vi "IO.vi"() -> ()   [LabVIEW 2024]
panel:
  in  "IO 16":bool
  in  "IO 15":bool
  in  "IO 14":bool
  in  "IO 13":bool
  in  "IO 12":bool
  in  "IO 11":bool
  in  "IO 10":bool
  in  "IO 9":bool
  in  "IO 8":bool
  in  "IO 7":bool
  in  "IO 6":bool
  in  "IO 5":bool
  in  "IO 4":bool
  in  "IO 3":bool
  in  "IO 2":bool
  in  "IO 1":bool
  out "IP":string="192.168.149.128"
  out "Port":dbl
  in  "Send":bool
  # "IO Light Control"
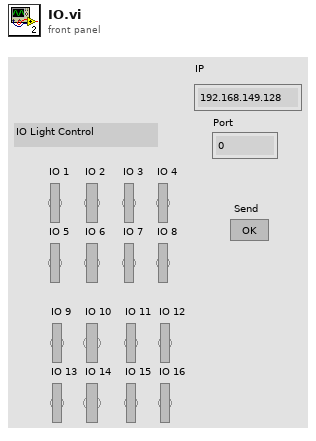
[diagram p1: front panel]
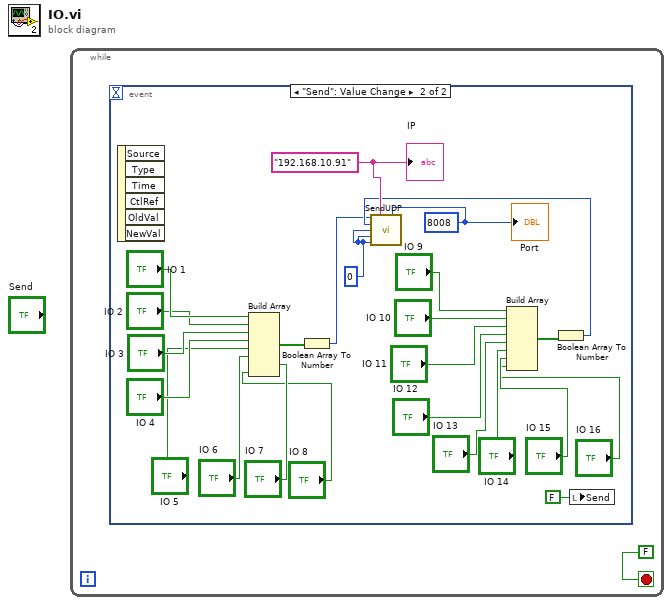
[diagram p0: block diagram]
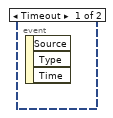
[diagram p2: hidden frame]
diagram:
  n1 = while {
    stop <- FALSE stop-if-true
    n2 = event shown="[1] \"Send\": Value Change" {
      selector: _ -> [_ _]
      dyn-events: _ -> [_ _]
      timeout: _ -> [_ _]
      event Timeout {
        n3 = event-data() -> ()  [unwired: 1 in, 3 out]
      }
      event "Send": Value Change {
        w6 = 0
        w24 = "192.168.10.91"
        w23 = 8008
        n4 = event-data() -> ()  [unwired: 1 in, 6 out]
        n5 = Build Array("IO 1", "IO 2", "IO 3", "IO 4", "IO 5", "IO 6", "IO 7", "IO 8") -> (w3:bool[])
        n6 = Boolean Array To Number(Boolean array=w3) -> (number=w2:u32)
        n7 = Build Array("IO 9", "IO 10", "IO 11", "IO 12", "IO 13", "IO 14", "IO 15", "IO 16") -> (w5:bool[])
        n8 = Boolean Array To Number(Boolean array=w5) -> (number=w4:u32)
        n9 = call "SendUDP.vi"("Arg3"=w2, "IP"=w24, "Port"=w23, "Arg4"=w4, "Arg5"=w6, "Arg6"=w6, "Arg7"=w6) -> ()  [unwired: 9 in]
        n10 = local write "Send"(FALSE ("Send")) -> ()
        "Port" <- w23
        "IP" <- w24
      }
    }
  }
